vi "[ce] Eval X-Y(a,t).vi"(6 "parameters":cluster{"name":string, "value":dbl}[](array[cluster]) {"value" format="%.2f"}, 7 "# points":u32=100, 8 "error in":errorcluster, 9 "formulas info":T1={"formula 1"="", "formula 2"="", "variable"="t"}, 10 "end":dbl=1.0 format="%.2f", 11 "start":dbl format="%.2f") -> (0 "error out":errorcluster, 1 "ticks":u32, 2 "Y":dbl[](array[numeric]) format="%.2f", 3 "X":dbl[](array[numeric]) format="%.2f")   [LabVIEW 2021]
doc: "The VI calculates the values of a function ( <b>f(t), g(t)</b> ), where <b>t</b> runs over the specified interval. In addition, the VI allows specifying additional parameters and evaluating them in formulas.\n\n::: CalcExpress Toolkit :::\nCopyright (c) 2000-2026 Konstantin Shifershteyn. All rights reserved."
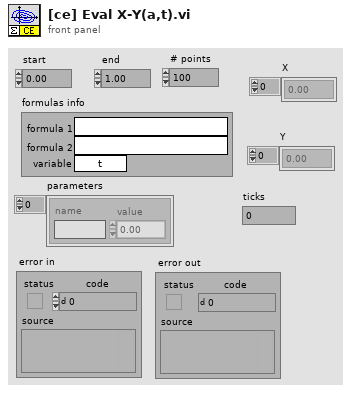
[diagram p1: front panel]
types:
  T1 = cluster{"formula 1":string, "formula 2":string, "variable":string}
  T2 = enum16{"create", "destroy", "set value", "get value"}
  T3 = typedef "VarMan Variable Context Handle.ctl" = i32
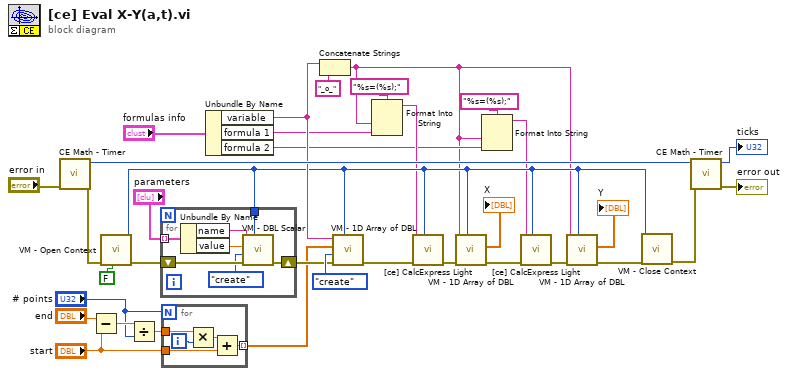
[diagram p0: block diagram]
diagram:
  n1 = call "CE Math - Timer.vi"("error in (no error)"="error in") -> ("error out"=w34:errorcluster, "ticks out"=w35:u32)  [unwired: 7 in]
  n2 = Subtract(x="end", y="start") -> (x-y=w23:dbl)
  n3 = call "VM - Open Context.vi"("close loose contexts (F)"=FALSE ("close loose contexts (T)"), "error in"=w34) -> ("error out"=w30:errorcluster, "VC Handle out"=w9:T3)  [unwired: 7 in, 1 out]
  n4 = Divide(x=w23, y="# points") -> (x/y=w24:dbl)
  n5 = for {
    shift-right: [w39] -> w18
    shift-left: w30 -> [w40]
    tunnel: "parameters" -> [w37] mode=indexing
    tunnel: w9 -> [w36]
    n6 = Unbundle By Name(w37) -> ("name"=w41:string, "value"=w42:dbl)
    n7 = call "VM - DBL Scalar.vi"("VC Handle"=w36, "error in"=w40, "cmd"=T2."create", "value in"=w42, "name_spec"=w41) -> ("error out"=w39:errorcluster)  [unwired: 1 in, 5 out]
  }
  n8 = for {
    N: "# points" -> [_]
    tunnel: w24 -> [w47]
    tunnel: "start" -> [w44]
    tunnel: [w43] -> w12 mode=indexing
    i -> [w46]
    n9 = Multiply(x=w47, y=w46) -> (x*y=w45:dbl)
    n10 = Add(x=w45, y=w44) -> (x+y=w43:dbl)
  }
  n11 = Unbundle By Name("formulas info") -> ("variable"=w10:string, "formula 1"=w7:string, "formula 2"=w5:string)
  n12 = Concatenate Strings(w10, "_o_" ("Substring")) -> (w4:string)
  n13 = call "VM - 1D Array of DBL.vi"("VC Handle"=w9, "error in"=w18, "cmd"=T2."create", "value in"=w12, "name_spec"=w10) -> ("error out"=w26:errorcluster)  [unwired: 1 in, 5 out]
  n14 = Format Into String(format string="%s=(%s);" ("Format String"), w4, w7) -> (resulting string=w6:string)  [unwired: 2 in, 1 out]
  n15 = call "[ce] CalcExpress Light.vi"("VC Handle"=w9, "error in"=w26, "expression"=w6) -> ("error out"=w25:errorcluster)  [unwired: 6 in, 2 out]
  n16 = call "VM - 1D Array of DBL.vi"("VC Handle"=w9, "error in"=w25, "name_spec"=w4) -> ("error out"=w16:errorcluster, "value out"=→"X":dbl[])  [unwired: 3 in, 4 out]
  n17 = Format Into String(format string="%s=(%s);" ("Format String"), w4, w5) -> (resulting string=w3:string)  [unwired: 2 in, 1 out]
  n18 = call "[ce] CalcExpress Light.vi"("VC Handle"=w9, "error in"=w16, "expression"=w3) -> ("error out"=w17:errorcluster)  [unwired: 6 in, 2 out]
  n19 = call "VM - 1D Array of DBL.vi"("VC Handle"=w9, "error in"=w17, "name_spec"=w4) -> ("error out"=w15:errorcluster, "value out"=→"Y":dbl[])  [unwired: 3 in, 4 out]
  n20 = call "VM - Close Context.vi"("error in"=w15, "VC Handle"=w9) -> ("error out"=w32:errorcluster)  [unwired: 8 in, 1 out]
  n21 = call "CE Math - Timer.vi"("error in (no error)"=w32, "ticks in"=w35) -> ("error out"=→"error out":errorcluster, "ticks out"=→"ticks":u32)  [unwired: 6 in]
